vi "SC Get Robot Project.vi"(8 "error in (no error)":errorcluster, 9 "target":string, 10 "window title":string="Open Deployed Project") -> (0 "error out":errorcluster, 1 "root":string, 2 "name":string, 3 "chosen?":bool)   [LabVIEW 2023]
doc: "Asks the robot (target, or this robot when empty) which projects it keeps. With several, the user chooses one (the one it runs is selected first and bold; italics: no local copy); with one, that one. Returns its root commit and name, both empty when the robot doesn't list projects. chosen? is false when the user cancels or the robot can't be asked (the tool's message is shown)."
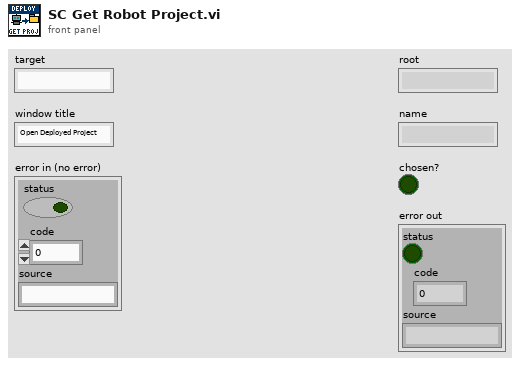
[diagram p1: front panel]
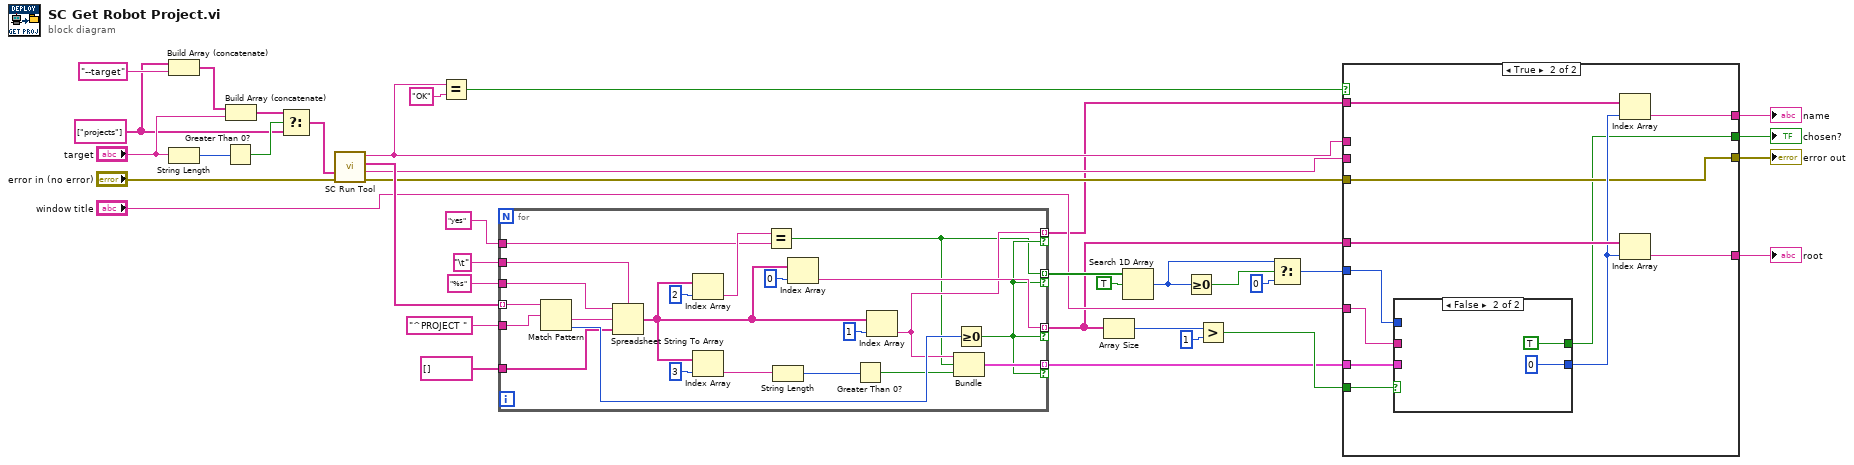
[diagram p0: block diagram]
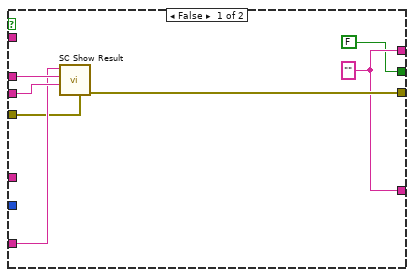
[diagram p2: hidden frame]
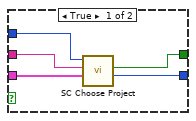
[diagram p3: hidden frame]
diagram:
  w31 = string[] ["projects"]
  n1 = Build Array (concatenate)(w31, "--target") -> (w36:string[])
  n2 = String Length(string="target") -> (length=w34:i32)
  n3 = Greater Than 0?(x=w34) -> (x > 0?=w33:bool)
  n4 = Build Array (concatenate)(w36, "target") -> (w32:string[])
  n5 = Select(t=w32, s=w33, f=w31) -> (s? t:f=w30:string[])
  n6 = call <vilib>:"SC Run Tool.vi"("error in (no error)"="error in (no error)", "arguments"=w30) -> ("error out"=w14:errorcluster, "output"=w13:string, "tool lines"=w28:string[], "result"=w12:string)  [unwired: 4 in, 2 out]
  n7 = Equal?(x=w12, y="OK") -> (x = y?=w1:bool)
  n8 = for {
    tunnel: w28 -> [w59] mode=indexing
    tunnel: "%s" -> [w56]
    tunnel: string[] [] -> [w54]
    tunnel: "\t" -> [w53]
    tunnel: "^PROJECT " -> [w58]
    tunnel: "yes" -> [w48]
    tunnel: [w42] -> w7 mode=indexing if=w39
    tunnel: [w41] -> w6 mode=indexing if=w39
    tunnel: [w40] -> w9 mode=indexing if=w39
    tunnel: [w38] -> w22 mode=indexing if=w39
    n9 = Match Pattern(string=w59, regular expression=w58) -> (after substring=w55:string, offset past match=w57:i32)  [unwired: 1 in, 2 out]
    n10 = Spreadsheet String To Array(delimiter (Tab)=w53, format string=w56, spreadsheet string=w55, array type (2D Dbl)=w54) -> (array=w47:string[])
    n11 = Index Array(array=w47, index=2) -> (element=w49:string)
    n12 = Index Array(array=w47, index=3) -> (element=w45:string)
    n13 = Equal?(x=w49, y=w48) -> (x = y?=w38:bool)
    n14 = String Length(string=w45) -> (length=w44:i32)
    n15 = Index Array(array=w47, index=0) -> (element=w42:string)
    n16 = Greater Than 0?(x=w44) -> (x > 0?=w43:bool)
    n17 = Index Array(array=w47, index=1) -> (element=w41:string)
    n18 = Bundle("String"=w41, w38, w43) -> (w40:cluster{"String":string, bool, bool})  [unwired: 1 in]
    n19 = Greater Or Equal To 0?(x=w57) -> (x >= 0?=w39:bool)
  }
  n20 = Array Size(array=w7) -> (size(s)=w17:i32)
  n21 = Search 1D Array(1D array=w22, element=TRUE) -> (index of element=w19:i32)  [unwired: 1 in]
  n22 = Greater Or Equal To 0?(x=w19) -> (x >= 0?=w20:bool)
  n23 = Greater?(x=w17, y=1) -> (0:w10:bool)
  n24 = Select(t=w19, s=w20, f=0) -> (s? t:f=w8:i32)
  n25 = case shown="True" w1 {
    tunnel: w14 -> [w63 w70]
    tunnel: w13 -> [w66 _]
    tunnel: w12 -> [w65 _]
    tunnel: "window title" -> [w64 w75]
    tunnel: w10 -> [_ w74]
    tunnel: w9 -> [_ w77]
    tunnel: w8 -> [_ w76]
    tunnel: w7 -> [_ w73]
    tunnel: w6 -> [_ w72]
    tunnel: [w62 w70] -> w5
    tunnel: [w61 w69] -> w4
    tunnel: [w61 w68] -> w3
    tunnel: [FALSE w67] -> w2
    frame False {
      w61 = ""
      n26 = call <vilib>:"SC Show Result.vi"("error in (no error)"=w63, "output"=w66, "result"=w65, "title"=w64) -> ("error out"=w62:errorcluster)  [unwired: 7 in]
    }
    frame True {
      n27 = case shown="False" w74 {
        tunnel: w77 -> [w82 _]
        tunnel: w76 -> [w81 _]
        tunnel: w75 -> [w80 _]
        tunnel: [w79 0] -> w71
        tunnel: [w78 TRUE] -> w67
        frame True {
          n28 = call "SC Choose Project.vi"("projects"=w82, "window title"=w80, "selected"=w81) -> ("index"=w79:i32, "chosen?"=w78:bool)  [unwired: 7 in]
        }
        frame False {
        }
      }
      n29 = Index Array(array=w72, index=w71) -> (element=w68:string)
      n30 = Index Array(array=w73, index=w71) -> (element=w69:string)
    }
  }
  "root" <- w4
  "name" <- w3
  "chosen?" <- w2
  "error out" <- w5
